vi "Util_Trajectory_WriteFile.vi"(4 "Trajectory is Cubic":bool, 5 "UseWeights":bool, 6 "Trajectory Is Relative":bool, 7 "TRAJECTORY_CONFIG":T1 {"End Velocity" format="%20.4f"; "StartVelocity" format="%20.4f"; "Max Acceleration" format="%20.4f"; "MaxVelocity" format="%20.4f"}, 8 "UtilityWayPoints":T2[](array[typedef]) {"WEIGHT" format="%13.3f"; "ANGLE" format="%13.3f"; "Y" format="%13.3f"; "X" format="%13.3f"}, 9 "TRAJECTORY":T3 {"States"."POSE"."ROTATION"."SIN" format="%13.4f"; "States"."POSE"."ROTATION"."COS" format="%13.4f"; "States"."POSE"."ROTATION"."VALUE" format="%13.4f"; "States"."POSE"."TRANSLATION"."Y" format="%14.3f"; "States"."POSE"."TRANSLATION"."X" format="%14.3f"; "TotalTImeSecs" format="%20.3f"}, 10 "Comment":string, 11 "Trajectory File Name":path) -> (0 "error out":errorcluster)   [LabVIEW 2019, in "Trajectory_Library.lvlib"]
doc: "Create a CSV file from a Trajectory data structure. This can be used on a PC or the RoboRIO.\n\nParameters:\n - Trajectory - Data structure containing trajectory\n - TrajectoryConfig - Trajectory configuration\n - Trajectory File Name - File name to write to. Existing files are overwritten.\n - Comment - Comment string to include in file comments.\n - Waypoints - waypoints to include in file comments\n - TrajectoryIsRelative - Relative if TRUE otherwise absolute\n - TrajectoryIsCubic - Cubic if TRUE otherwise Quintic\n\nReturns:\n - Error out - returned error cluster\n\nReturns:\n - outTrajectory - Trajectory data structure\n - Error out - returned error cluster"
uses:
  Trajectory_Library.lvlib
  TypeDef/TRAJECTORY.ctl
  TypeDef/TRAJ_STATE.ctl
  TypeDef/POSE2D.ctl
  TypeDef/TRANSLATION2D.ctl
  TypeDef/ROTATION2D.ctl
  TypeDef/DISPLAY_WEIGHTED_WAYPOINT.ctl
  TypeDef/TRAJ_CONFIG.ctl
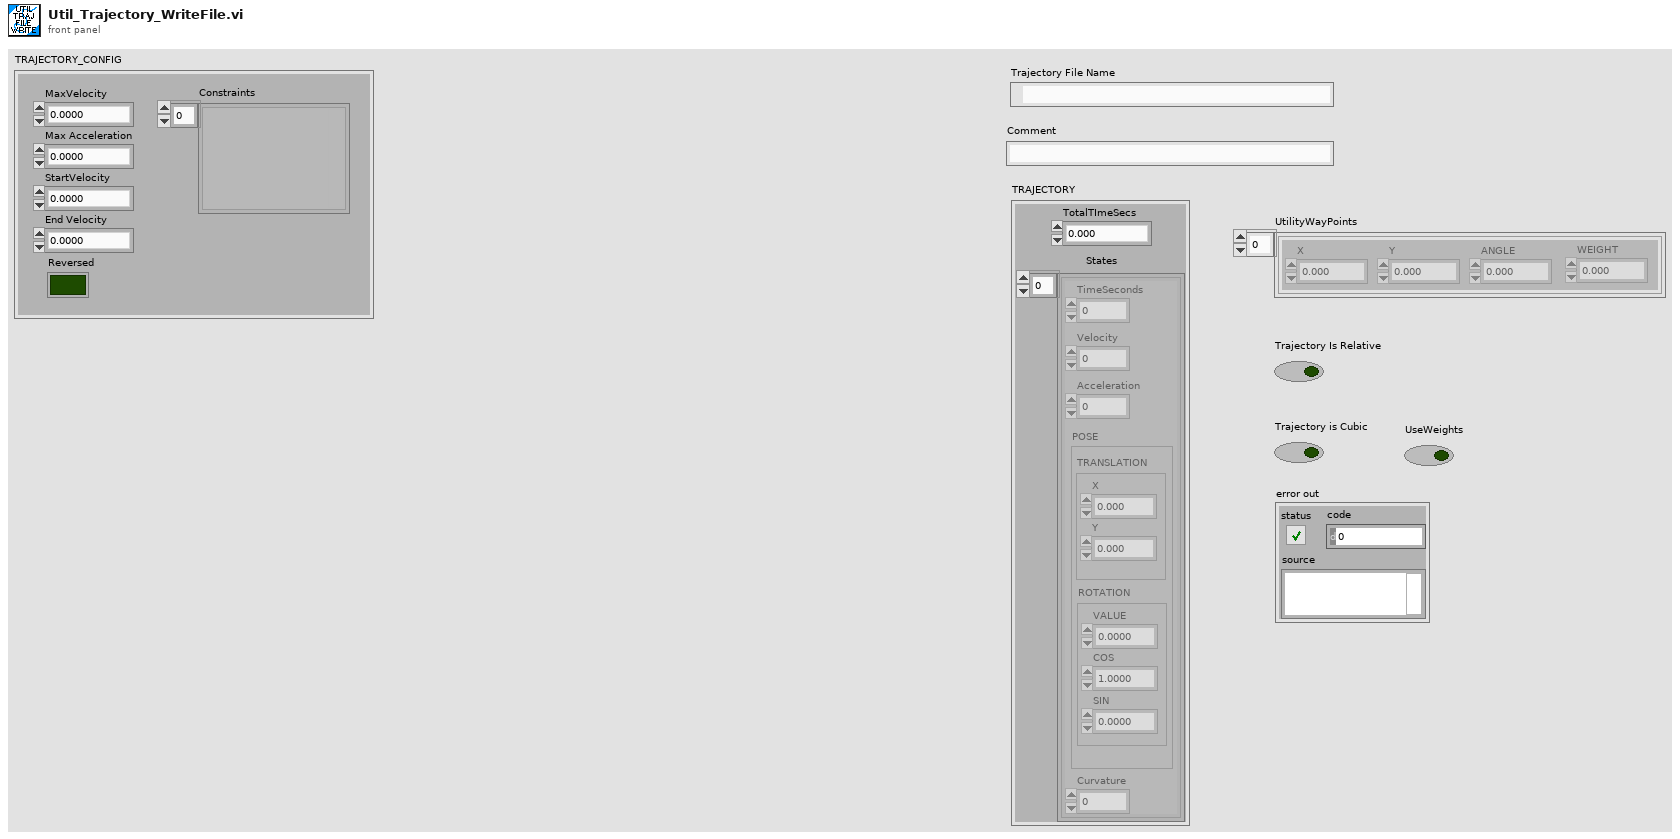
[diagram p1: front panel]
types:
  T1 = typedef "Trajectory_Library.lvlib/TRAJ_CONFIG.ctl" = cluster{"MaxVelocity":dbl, "Max Acceleration":dbl, "StartVelocity":dbl, "End Velocity":dbl, "Reversed":bool, "Constraints":variant[]}
  T2 = typedef "Trajectory_Library.lvlib/DISPLAY_WEIGHTED_WAYPOINT.ctl" = cluster{"X":dbl, "Y":dbl, "ANGLE":dbl, "WEIGHT":dbl}
  T3 = typedef "Trajectory_Library.lvlib/TRAJECTORY.ctl" = cluster{"TotalTImeSecs":dbl, "States":T4[]}
  T4 = typedef "Trajectory_Library.lvlib/TRAJ_STATE.ctl" = cluster{"TimeSeconds":dbl, "Velocity":dbl, "Acceleration":dbl, "POSE":T5, "Curvature":dbl}
  T5 = typedef "Trajectory_Library.lvlib/POSE2D.ctl" = cluster{"TRANSLATION":T6, "ROTATION":T7}
  T6 = typedef "Trajectory_Library.lvlib/TRANSLATION2D.ctl" = cluster{"X":dbl, "Y":dbl}
  T7 = typedef "Trajectory_Library.lvlib/ROTATION2D.ctl" = cluster{"VALUE":dbl, "COS":dbl, "SIN":dbl}
  T8 = enum16{"open", "replace", "create", "open or create", "replace or create", "replace or create with confirmation"}
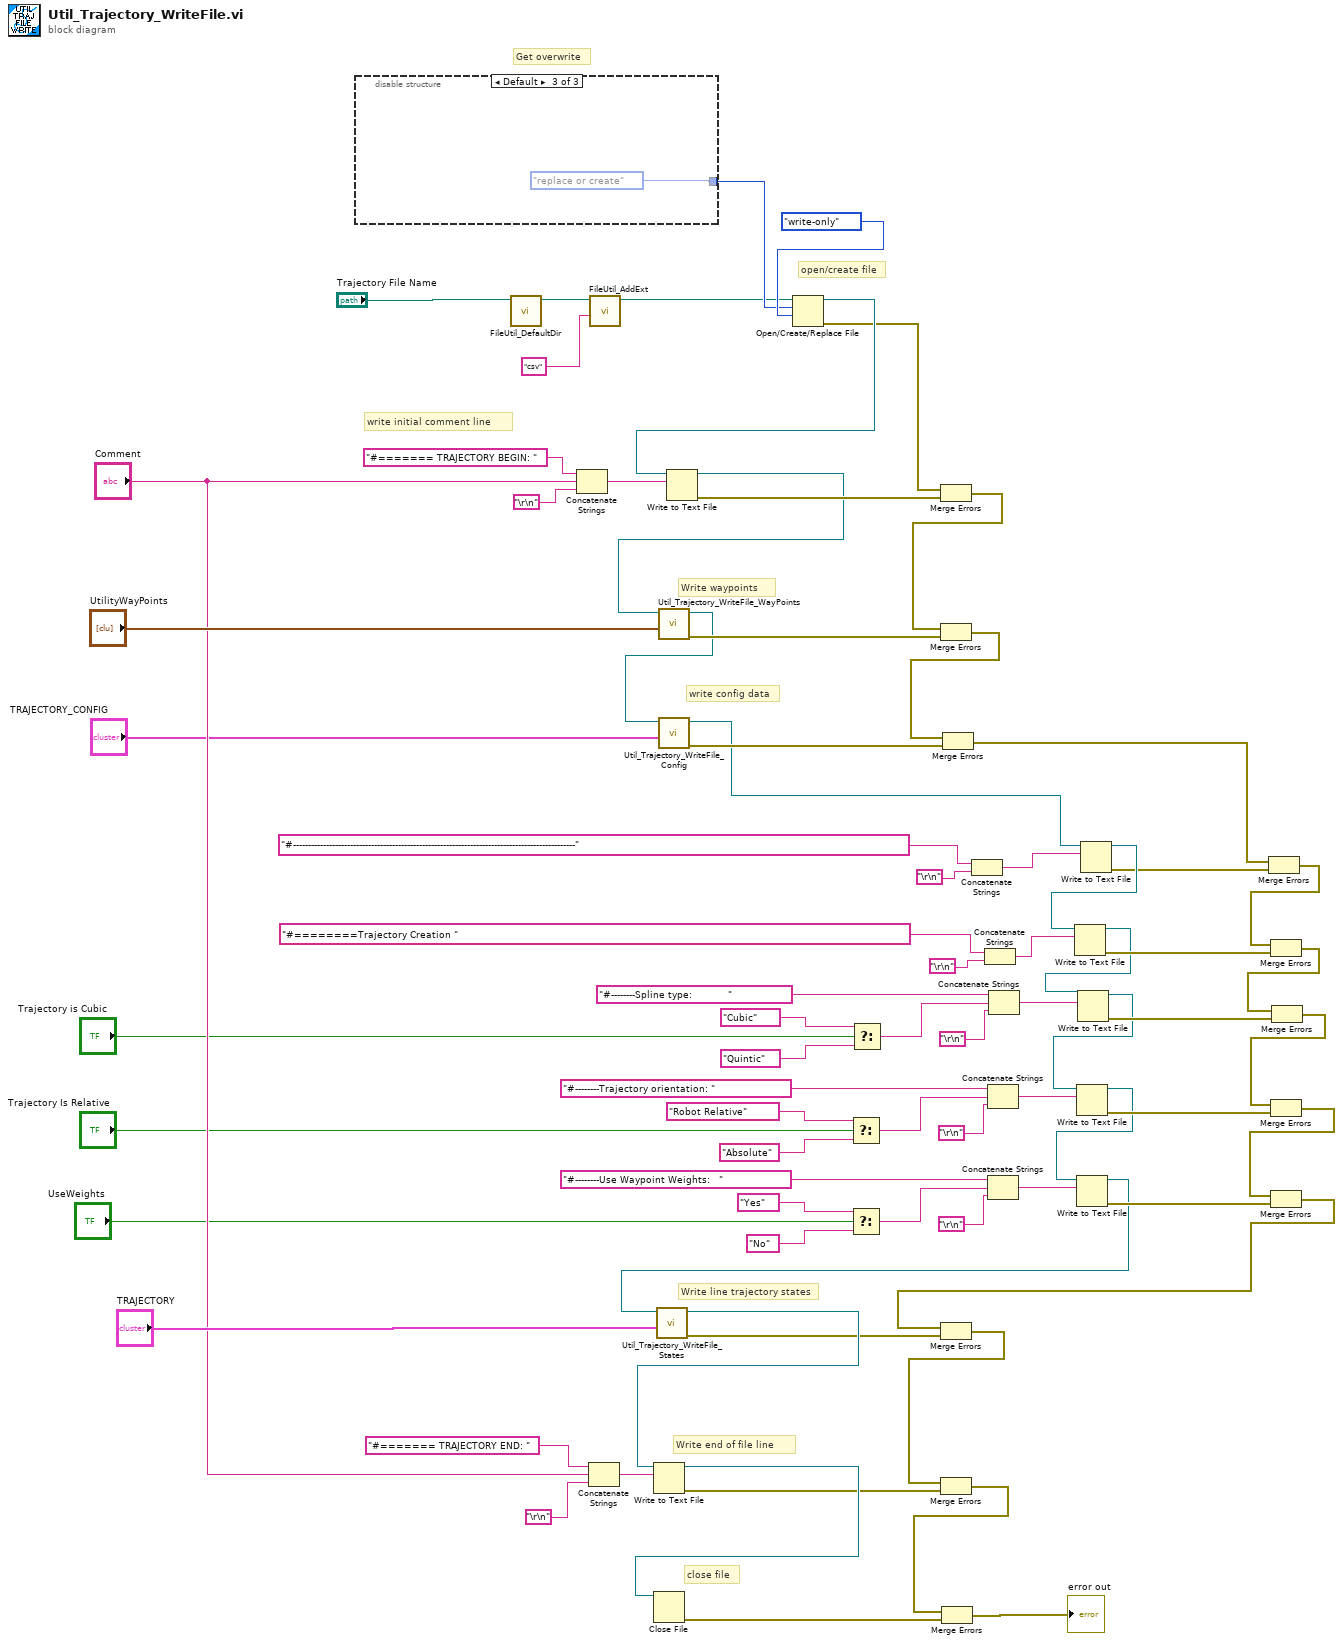
[diagram p0: block diagram]
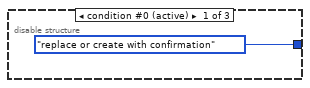
[diagram p2: hidden frame]
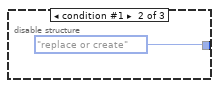
[diagram p3: hidden frame]
diagram:
  # "Get overwrite"
  # "write config data"
  # "Write line trajectory states"
  # "open/create file"
  # "Write waypoints"
  # "close file"
  # "Write end of file line"
  # "write initial comment line"
  n1 = disable-structure shown="Default" {
    disable-tunnel: [T8."replace or create with confirmation" ("operation (0:open)") T8."replace or create" ("operation (0:open)") T8."replace or create" ("operation (0:open)")] -> w5
    frame condition #0 (active) {
    }
    frame condition #1 {
    }
    frame condition #2 {
    }
  }
  n2 = call "FileUtil_DefaultDir.vi"("Path in"="Trajectory File Name") -> ("Path Out"=w4:path)  [unwired: 10 in]
  n3 = Concatenate Strings("#======= TRAJECTORY BEGIN: " ("string"), "Comment", "\r\n") -> (w76:string)
  n4 = Concatenate Strings("#======= TRAJECTORY END: " ("string"), "Comment", "\r\n") -> (w72:string)
  n5 = call "FileUtil_AddExt.vi"("Extension"="csv", "Path in"=w4) -> ("Path out"=w1:path)  [unwired: 9 in]
  n6 = Open/Create/Replace File(file path (use dialog)=w1, operation (0:open)=w5, access (0:read/write)=enum16{"read/write", "read-only", "write-only"}."write-only") -> (refnum out=w68:refnum<file>, error out=w63:errorcluster)  [unwired: 3 in, 1 out]
  n7 = Write to Text File(file (use dialog)=w68, text=w76) -> (refnum out=w54:refnum<file>, error out=w64:errorcluster)  [unwired: 2 in, 1 out]
  n8 = call "Util_Trajectory_WriteFile_WayPoints.vi"("UtilityWayPoints"="UtilityWayPoints", "Byte Steam File In"=w54) -> ("error out"=w62:errorcluster, "Byte Steam File Out"=w52:refnum<file>)  [unwired: 8 in]
  n9 = call "Util_Trajectory_WriteFile_Config.vi"("TRAJECTORY_CONFIG"="TRAJECTORY_CONFIG", "Byte Steam File In"=w52) -> ("error out"=w51:errorcluster, "Byte Steam File Out"=w32:refnum<file>)  [unwired: 8 in]
  n10 = Select(t="Robot Relative" ("string"), s="Trajectory Is Relative", f="Absolute" ("string")) -> (s? t:f=w40:string)
  n11 = Select(t="Yes" ("string"), s="UseWeights", f="No" ("string")) -> (s? t:f=w14:string)
  n12 = Select(t="Cubic" ("string"), s="Trajectory is Cubic", f="Quintic" ("string")) -> (s? t:f=w26:string)
  n13 = Merge Errors(w63, w64) -> (w55:errorcluster)
  n14 = Merge Errors(w55, w62) -> (w50:errorcluster)
  n15 = Merge Errors(w50, w51) -> (w30:errorcluster)
  n16 = Concatenate Strings("#----------------------------------------------------------------------------------------------" ("string"), "\r\n") -> (w44:string)
  n17 = Concatenate Strings("#========Trajectory Creation " ("string"), "\r\n") -> (w47:string)
  n18 = Concatenate Strings("#--------Trajectory orientation: " ("string"), w40, "\r\n") -> (w42:string)
  n19 = Concatenate Strings("#--------Use Waypoint Weights:   " ("string"), w14, "\r\n") -> (w16:string)
  n20 = Concatenate Strings("#--------Spline type:            " ("string"), w26, "\r\n") -> (w28:string)
  n21 = Write to Text File(file (use dialog)=w32, text=w44) -> (refnum out=w36:refnum<file>, error out=w34:errorcluster)  [unwired: 2 in, 1 out]
  n22 = Write to Text File(file (use dialog)=w36, text=w47) -> (refnum out=w22:refnum<file>, error out=w35:errorcluster)  [unwired: 2 in, 1 out]
  n23 = Write to Text File(file (use dialog)=w22, text=w28) -> (refnum out=w21:refnum<file>, error out=w27:errorcluster)  [unwired: 2 in, 1 out]
  n24 = Write to Text File(file (use dialog)=w21, text=w42) -> (refnum out=w8:refnum<file>, error out=w41:errorcluster)  [unwired: 2 in, 1 out]
  n25 = Write to Text File(file (use dialog)=w8, text=w16) -> (refnum out=w7:refnum<file>, error out=w15:errorcluster)  [unwired: 2 in, 1 out]
  n26 = call "Util_Trajectory_WriteFile_States.vi"("Trajectory"="TRAJECTORY", "Byte Steam File In"=w7) -> ("error out"=w61:errorcluster, "Byte Steam File Out"=w66:refnum<file>)  [unwired: 8 in]
  n27 = Write to Text File(file (use dialog)=w66, text=w72) -> (refnum out=w65:refnum<file>, error out=w59:errorcluster)  [unwired: 2 in, 1 out]
  n28 = Close File(refnum=w65) -> (error out=w58:errorcluster)  [unwired: 1 in, 1 out]
  n29 = Merge Errors(w30, w34) -> (w33:errorcluster)
  n30 = Merge Errors(w33, w35) -> (w20:errorcluster)
  n31 = Merge Errors(w20, w27) -> (w19:errorcluster)
  n32 = Merge Errors(w19, w41) -> (w10:errorcluster)
  n33 = Merge Errors(w10, w15) -> (w9:errorcluster)
  n34 = Merge Errors(w9, w61) -> (w60:errorcluster)
  n35 = Merge Errors(w60, w59) -> (w57:errorcluster)
  n36 = Merge Errors(w57, w58) -> (→"error out":errorcluster)
